vi "RemoteVI Arrange Controls.vi"(0 "VI":refnum<vi>, 5 "layout":T1(array[cluster]), 7 "panel size":cluster{"width":i32, "height":i32}, 9 "title":string) -> ()   [LabVIEW 2020, in "RemoteVI.lvlib"]
doc: "Lays out a running VI's own front panel (the RemoteVI UIs arrange themselves when they start: AIXML has no panel layout): every top-level control whose label is in layout is moved to left, top (Position, label included) and sized to width, height where LabVIEW lets a running VI resize it (a boolean: Button Size; a string: Size; a multicolumn listbox: as many rows as fit into height - 0 keeps the size); a NEGATIVE width hides the control instead (Visible FALSE; the RemoteVI UIs hide their tick and stop controls so); the window gets title and a panel area of panel size (Front Panel Window:Panel Bounds, its top-left kept). A boolean shows its label as its boolean text (centred) instead of beside it, so it looks like a labelled button. Controls not in layout are left where they are. The tool bar, menu bar and scroll bars are hidden (where LabVIEW allows it while the VI runs). Errors of the property writes are ignored; the panel still opens."
uses:
  RemoteVI.lvlib
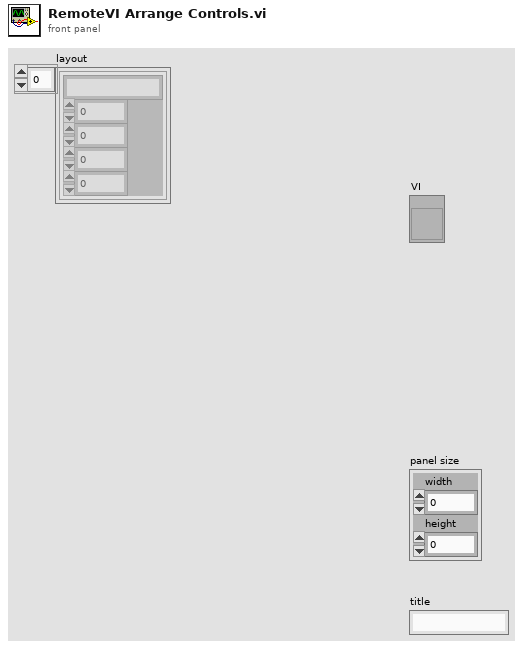
[diagram p1: front panel]
types:
  T1 = cluster{"label":string, "left":i32, "top":i32, "width":i32, "height":i32}[]
  T2 = typedef "LVPositionTypeDef.ctl" = cluster{"Left":i32, "Top":i32}
  T3 = cluster{"label":string, "left":i32, "top":i32, "width":i32, "height":i32}
  T4 = typedef "LVRectTypeDef.ctl" = cluster{"left":i16, "top":i16, "right":i16, "bottom":i16}
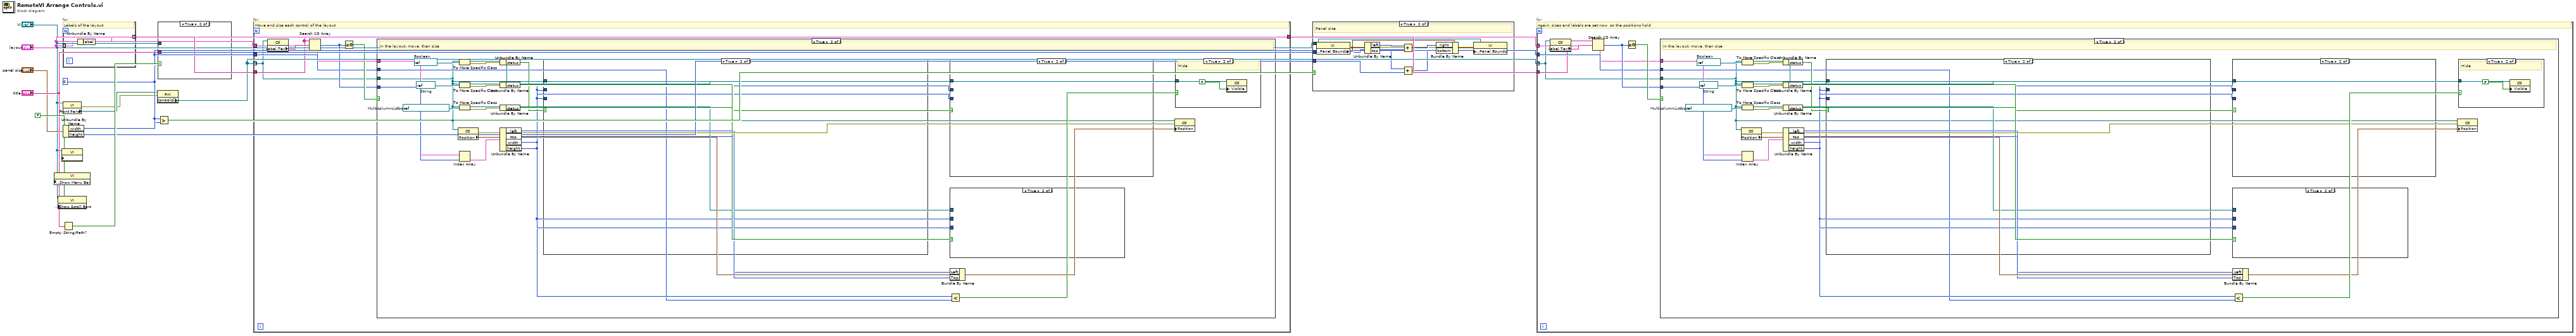
[diagram p0: block diagram]
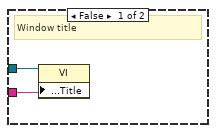
[diagram p2: hidden frame]
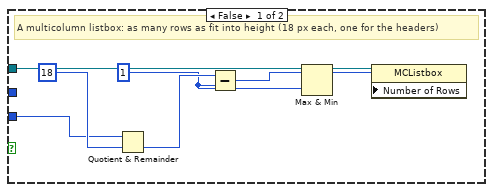
[diagram p6: hidden frame]
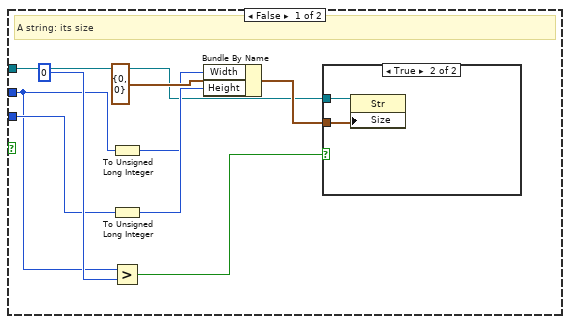
[diagram p7: hidden frame]
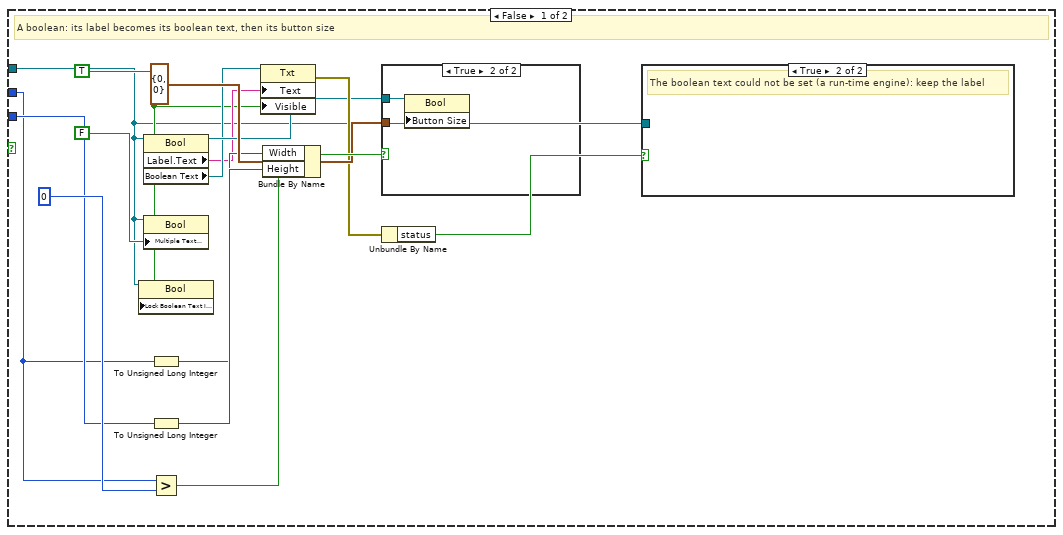
[diagram p9: hidden frame]
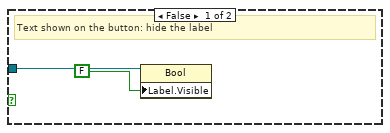
[diagram p11: hidden frame]
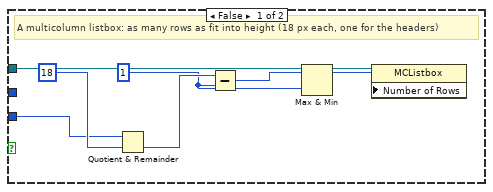
[diagram p14: hidden frame]
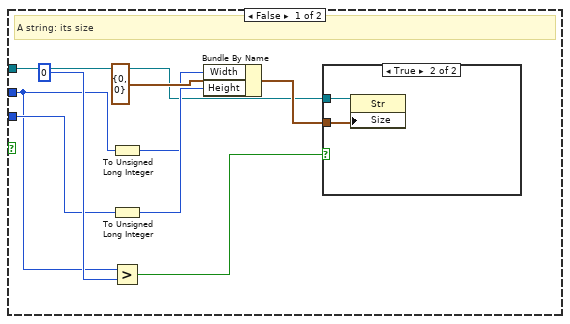
[diagram p15: hidden frame]
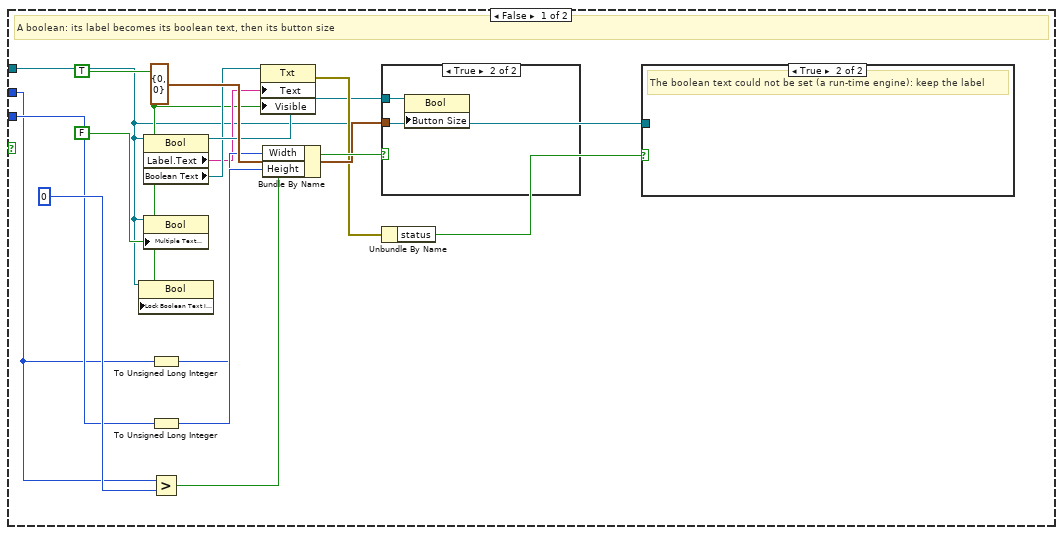
[diagram p17: hidden frame]
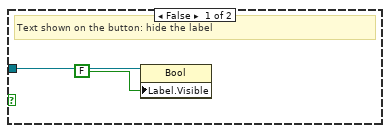
[diagram p19: hidden frame]
diagram:
  w14 = FALSE
  w9 = 0
  n1 = property class="VI"(reference="VI", "Front Panel Window:Show Menu Bar"=w14) -> ()  [unwired: 1 in, 2 out]
  n2 = property class="VI"(reference="VI", "Front Panel Window:Show Scroll Bars"=w14) -> ()  [unwired: 1 in, 2 out]
  n3 = property class="VI"(reference="VI", "Tool Bar:Visible"=w14) -> ()  [unwired: 1 in, 2 out]
  n4 = for {
    tunnel: "layout" -> [w16] mode=indexing
    tunnel: [w17] -> w8 mode=indexing
    # "Labels of the layout"
    n5 = Unbundle By Name(w16) -> ("label"=w17:string)
  }
  n6 = property class="VI"(reference="VI") -> (error out=w5:errorcluster, "Front Panel"=w6:refnum<vi>)  [unwired: 1 in, 1 out]
  n7 = Unbundle By Name("panel size") -> ("width"=w11:i32, "height"=w12:i32)
  n8 = Empty String/Path?(string/path="title") -> (empty?=w15:bool)
  n9 = property class="Pnl"(reference=w6, error in=w5) -> ("Controls[]"=w7:refnum<vi>[])  [unwired: 2 out]
  n10 = case shown="True" w15 {
    tunnel: "VI" -> [w18 _]
    tunnel: "title" -> [w19 _]
    frame False {
      # "Window title"
      n11 = property class="VI"(reference=w18, "Front Panel Window:Title"=w19) -> ()  [unwired: 1 in, 2 out]
    }
    frame True {
    }
  }
  n12 = Greater?(x=w11, y=w9) -> (0:w13:bool)
  n13 = for {
    tunnel: "layout" -> [w22]
    tunnel: w9 -> [w23]
    tunnel: w7 -> [w20] mode=indexing
    tunnel: w8 -> [w21]
    tunnel: [w21] -> w10
    # "Move and size each control of the layout"
    n14 = property class="Ctl"(reference=w20) -> ("Label.Text"=w24:string)  [unwired: 1 in, 2 out]
    n15 = Search 1D Array(1D array=w21, element=w24) -> (index of element=w25:i32)  [unwired: 1 in]
    n16 = Greater Or Equal To 0?(x=w25) -> (x >= 0?=w26:bool)
    n17 = case shown="True" w26 {
      tunnel: w22 -> [_ w28]
      tunnel: w23 -> [_ w30]
      tunnel: w20 -> [_ w27]
      tunnel: w25 -> [_ w29]
      frame False {
      }
      frame True {
        w44 = refnum<vi> refnum  # MulticolumnListbox
        w40 = refnum<vi> refnum  # String
        w36 = refnum<vi> refnum  # Boolean
        # "In the layout: move, then size"
        n18 = property class="Ctl"(reference=w27) -> (error out=w49:errorcluster, "Position"=w48:T2)  [unwired: 1 in, 1 out]
        n19 = To More Specific Class(target class=w36, reference=w27) -> (specific class reference=w37:refnum<vi>, error out=w38:errorcluster)  [unwired: 1 in]
        n20 = To More Specific Class(target class=w40, reference=w27) -> (specific class reference=w41:refnum<vi>, error out=w42:errorcluster)  [unwired: 1 in]
        n21 = To More Specific Class(target class=w44, reference=w27) -> (specific class reference=w45:refnum<vi>, error out=w46:errorcluster)  [unwired: 1 in]
        n22 = Index Array(array=w28, index=w29) -> (element=w31:T3)
        n23 = Unbundle By Name(w38) -> ("status"=w39:bool)
        n24 = Unbundle By Name(w42) -> ("status"=w43:bool)
        n25 = Unbundle By Name(w46) -> ("status"=w47:bool)
        n26 = Unbundle By Name(w31) -> ("left"=w32:i32, "top"=w33:i32, "width"=w34:i32, "height"=w35:i32)
        n27 = case shown="True" w39 {
          tunnel: w37 -> [w72 _]
          tunnel: w34 -> [w73 _]
          tunnel: w35 -> [w74 _]
          frame False {
            w75 = TRUE
            # "A boolean: its label becomes its boolean text, then its button size"
            n28 = property class="Bool"(reference=w72, "Lock Boolean Text In Center"=w75) -> ()  [unwired: 1 in, 2 out]
            n29 = property class="Bool"(reference=w72) -> (reference out=w79:refnum<vi>, "Label.Text"=w77:string, "Boolean Text"=w78:refnum<vi>)  [unwired: 1 in, 1 out]
            n30 = property class="Bool"(reference=w72, "Multiple Text String"=FALSE) -> ()  [unwired: 1 in, 2 out]
            n31 = To Unsigned Long Integer(number=w73) -> (unsigned 32bit integer=w82:u32)
            n32 = To Unsigned Long Integer(number=w74) -> (unsigned 32bit integer=w83:u32)
            n33 = Greater?(x=w73, y=0) -> (0:w87:bool)
            n34 = property class="Txt"(reference=w78, "Text"=w77, "Visible"=w75) -> (error out=w80:errorcluster)  [unwired: 1 in, 1 out]
            n35 = Bundle By Name(cluster=cluster{"Width":u32, "Height":u32} {"Width"=0, "Height"=0}, "Width"=w82, "Height"=w83) -> (w85:cluster{"Width":u32, "Height":u32})
            n36 = case shown="True" w87 {
              tunnel: w79 -> [_ w88]
              tunnel: w85 -> [_ w89]
              frame False {
              }
              frame True {
                n37 = property class="Bool"(reference=w88, "Button Size"=w89) -> ()  [unwired: 1 in, 2 out]
              }
            }
            n38 = Unbundle By Name(w80) -> ("status"=w81:bool)
            n39 = case shown="True" w81 {
              tunnel: w72 -> [w90 _]
              frame False {
                # "Text shown on the button: hide the label"
                n40 = property class="Bool"(reference=w90, "Label.Visible"=FALSE) -> ()  [unwired: 1 in, 2 out]
              }
              frame True {
                # "The boolean text could not be set (a run-time engine): keep the label"
              }
            }
          }
          frame True {
          }
        }
        n41 = case shown="True" w43 {
          tunnel: w41 -> [w61 _]
          tunnel: w34 -> [w62 _]
          tunnel: w35 -> [w63 _]
          frame False {
            # "A string: its size"
            n42 = To Unsigned Long Integer(number=w62) -> (unsigned 32bit integer=w64:u32)
            n43 = To Unsigned Long Integer(number=w63) -> (unsigned 32bit integer=w65:u32)
            n44 = Greater?(x=w62, y=0) -> (0:w69:bool)
            n45 = Bundle By Name(cluster=cluster{"Width":u32, "Height":u32} {"Width"=0, "Height"=0}, "Width"=w64, "Height"=w65) -> (w67:cluster{"Width":u32, "Height":u32})
            n46 = case shown="True" w69 {
              tunnel: w61 -> [_ w70]
              tunnel: w67 -> [_ w71]
              frame False {
              }
              frame True {
                n47 = property class="Str"(reference=w70, "Size"=w71) -> ()  [unwired: 1 in, 2 out]
              }
            }
          }
          frame True {
          }
        }
        n48 = case shown="True" w47 {
          tunnel: w45 -> [w54 _]
          tunnel: w34 -> [_ _]
          tunnel: w35 -> [w55 _]
          frame False {
            w57 = 1
            # "A multicolumn listbox: as many rows as fit into height (18 px each, one for the headers)"
            n49 = Quotient & Remainder(x=w55, y=18) -> (floor(x/y)=w58:i32)  [unwired: 1 out]
            n50 = Subtract(x=w58, y=w57) -> (x-y=w59:i32)
            n51 = Max & Min(x=w59, y=w57) -> (max(x,y)=w60:i32)  [unwired: 1 out]
            n52 = property class="MCListbox"(reference=w54, "Number of Rows"=w60) -> ()  [unwired: 1 in, 2 out]
          }
          frame True {
          }
        }
        n53 = Bundle By Name(cluster=w48, "Left"=w32, "Top"=w33) -> (w50:T2)
        n54 = Less?(x=w34, y=w30) -> (x < y?=w51:bool)
        n55 = property class="Ctl"(reference=w27, error in=w49, "Position"=w50) -> ()  [unwired: 2 out]
        n56 = case shown="True" w51 {
          tunnel: w27 -> [_ w52]
          frame False {
          }
          frame True {
            # "Hide"
            n57 = property class="Ctl"(reference=w52, "Visible"=FALSE) -> ()  [unwired: 1 in, 2 out]
          }
        }
      }
    }
  }
  n58 = case shown="True" w13 {
    tunnel: "VI" -> [_ w92]
    tunnel: w11 -> [_ w93]
    tunnel: w12 -> [_ w94]
    frame False {
    }
    frame True {
      # "Panel size"
      n59 = property class="VI"(reference=w92) -> (error out=w95:errorcluster, "Front Panel Window:Panel Bounds"=w96:T4)  [unwired: 1 in, 1 out]
      n60 = Unbundle By Name(w96) -> ("left"=w97:i16, "top"=w98:i16)
      n61 = Add(x=w97, y=w93) -> (x+y=w99:i32)
      n62 = Add(x=w98, y=w94) -> (x+y=w100:i32)
      n63 = Bundle By Name(cluster=w96, "right"=w99, "bottom"=w100) -> (w101:T4)
      n64 = property class="VI"(reference=w92, error in=w95, "Front Panel Window:Panel Bounds"=w101) -> ()  [unwired: 2 out]
    }
  }
  n65 = for {
    tunnel: "layout" -> [w104]
    tunnel: w9 -> [w105]
    tunnel: w7 -> [w102] mode=indexing
    tunnel: w10 -> [w103]
    # "Again: sizes and labels are set now, so the positions hold"
    n66 = property class="Ctl"(reference=w102) -> ("Label.Text"=w106:string)  [unwired: 1 in, 2 out]
    n67 = Search 1D Array(1D array=w103, element=w106) -> (index of element=w107:i32)  [unwired: 1 in]
    n68 = Greater Or Equal To 0?(x=w107) -> (x >= 0?=w108:bool)
    n69 = case shown="True" w108 {
      tunnel: w104 -> [_ w110]
      tunnel: w105 -> [_ w112]
      tunnel: w102 -> [_ w109]
      tunnel: w107 -> [_ w111]
      frame False {
      }
      frame True {
        w126 = refnum<vi> refnum  # MulticolumnListbox
        w122 = refnum<vi> refnum  # String
        w118 = refnum<vi> refnum  # Boolean
        # "In the layout: move, then size"
        n70 = property class="Ctl"(reference=w109) -> (error out=w131:errorcluster, "Position"=w130:T2)  [unwired: 1 in, 1 out]
        n71 = To More Specific Class(target class=w118, reference=w109) -> (specific class reference=w119:refnum<vi>, error out=w120:errorcluster)  [unwired: 1 in]
        n72 = To More Specific Class(target class=w122, reference=w109) -> (specific class reference=w123:refnum<vi>, error out=w124:errorcluster)  [unwired: 1 in]
        n73 = To More Specific Class(target class=w126, reference=w109) -> (specific class reference=w127:refnum<vi>, error out=w128:errorcluster)  [unwired: 1 in]
        n74 = Index Array(array=w110, index=w111) -> (element=w113:T3)
        n75 = Unbundle By Name(w120) -> ("status"=w121:bool)
        n76 = Unbundle By Name(w124) -> ("status"=w125:bool)
        n77 = Unbundle By Name(w128) -> ("status"=w129:bool)
        n78 = Unbundle By Name(w113) -> ("left"=w114:i32, "top"=w115:i32, "width"=w116:i32, "height"=w117:i32)
        n79 = case shown="True" w121 {
          tunnel: w119 -> [w154 _]
          tunnel: w116 -> [w155 _]
          tunnel: w117 -> [w156 _]
          frame False {
            w157 = TRUE
            # "A boolean: its label becomes its boolean text, then its button size"
            n80 = property class="Bool"(reference=w154, "Lock Boolean Text In Center"=w157) -> ()  [unwired: 1 in, 2 out]
            n81 = property class="Bool"(reference=w154) -> (reference out=w161:refnum<vi>, "Label.Text"=w159:string, "Boolean Text"=w160:refnum<vi>)  [unwired: 1 in, 1 out]
            n82 = property class="Bool"(reference=w154, "Multiple Text String"=FALSE) -> ()  [unwired: 1 in, 2 out]
            n83 = To Unsigned Long Integer(number=w155) -> (unsigned 32bit integer=w164:u32)
            n84 = To Unsigned Long Integer(number=w156) -> (unsigned 32bit integer=w165:u32)
            n85 = Greater?(x=w155, y=0) -> (0:w169:bool)
            n86 = property class="Txt"(reference=w160, "Text"=w159, "Visible"=w157) -> (error out=w162:errorcluster)  [unwired: 1 in, 1 out]
            n87 = Bundle By Name(cluster=cluster{"Width":u32, "Height":u32} {"Width"=0, "Height"=0}, "Width"=w164, "Height"=w165) -> (w167:cluster{"Width":u32, "Height":u32})
            n88 = case shown="True" w169 {
              tunnel: w161 -> [_ w170]
              tunnel: w167 -> [_ w171]
              frame False {
              }
              frame True {
                n89 = property class="Bool"(reference=w170, "Button Size"=w171) -> ()  [unwired: 1 in, 2 out]
              }
            }
            n90 = Unbundle By Name(w162) -> ("status"=w163:bool)
            n91 = case shown="True" w163 {
              tunnel: w154 -> [w172 _]
              frame False {
                # "Text shown on the button: hide the label"
                n92 = property class="Bool"(reference=w172, "Label.Visible"=FALSE) -> ()  [unwired: 1 in, 2 out]
              }
              frame True {
                # "The boolean text could not be set (a run-time engine): keep the label"
              }
            }
          }
          frame True {
          }
        }
        n93 = case shown="True" w125 {
          tunnel: w123 -> [w143 _]
          tunnel: w116 -> [w144 _]
          tunnel: w117 -> [w145 _]
          frame False {
            # "A string: its size"
            n94 = To Unsigned Long Integer(number=w144) -> (unsigned 32bit integer=w146:u32)
            n95 = To Unsigned Long Integer(number=w145) -> (unsigned 32bit integer=w147:u32)
            n96 = Greater?(x=w144, y=0) -> (0:w151:bool)
            n97 = Bundle By Name(cluster=cluster{"Width":u32, "Height":u32} {"Width"=0, "Height"=0}, "Width"=w146, "Height"=w147) -> (w149:cluster{"Width":u32, "Height":u32})
            n98 = case shown="True" w151 {
              tunnel: w143 -> [_ w152]
              tunnel: w149 -> [_ w153]
              frame False {
              }
              frame True {
                n99 = property class="Str"(reference=w152, "Size"=w153) -> ()  [unwired: 1 in, 2 out]
              }
            }
          }
          frame True {
          }
        }
        n100 = case shown="True" w129 {
          tunnel: w127 -> [w136 _]
          tunnel: w116 -> [_ _]
          tunnel: w117 -> [w137 _]
          frame False {
            w139 = 1
            # "A multicolumn listbox: as many rows as fit into height (18 px each, one for the headers)"
            n101 = Quotient & Remainder(x=w137, y=18) -> (floor(x/y)=w140:i32)  [unwired: 1 out]
            n102 = Subtract(x=w140, y=w139) -> (x-y=w141:i32)
            n103 = Max & Min(x=w141, y=w139) -> (max(x,y)=w142:i32)  [unwired: 1 out]
            n104 = property class="MCListbox"(reference=w136, "Number of Rows"=w142) -> ()  [unwired: 1 in, 2 out]
          }
          frame True {
          }
        }
        n105 = Bundle By Name(cluster=w130, "Left"=w114, "Top"=w115) -> (w132:T2)
        n106 = Less?(x=w116, y=w112) -> (x < y?=w133:bool)
        n107 = property class="Ctl"(reference=w109, error in=w131, "Position"=w132) -> ()  [unwired: 2 out]
        n108 = case shown="True" w133 {
          tunnel: w109 -> [_ w134]
          frame False {
          }
          frame True {
            # "Hide"
            n109 = property class="Ctl"(reference=w134, "Visible"=FALSE) -> ()  [unwired: 1 in, 2 out]
          }
        }
      }
    }
  }
